vi "VIH HelpGen - Write HTML File - Common - Owning Palette.vi"(5 "HTML Folder":path, 8 "error in":errorcluster, 10 "Owning Palette":cluster{"Name":string, "HTML Path":path}, 11 "HTML in":string) -> (0 "error out":errorcluster, 3 "HTML out":string)   [LabVIEW 2014]
doc: "::: VI Helpeks :::\nCopyright (c) 2000-2026 Konstantin Shifershteyn. All rights reserved."
panel:
  # "VI Helpeks\nCopyright (c) 2012-2026 Konstantin Shifershteyn"
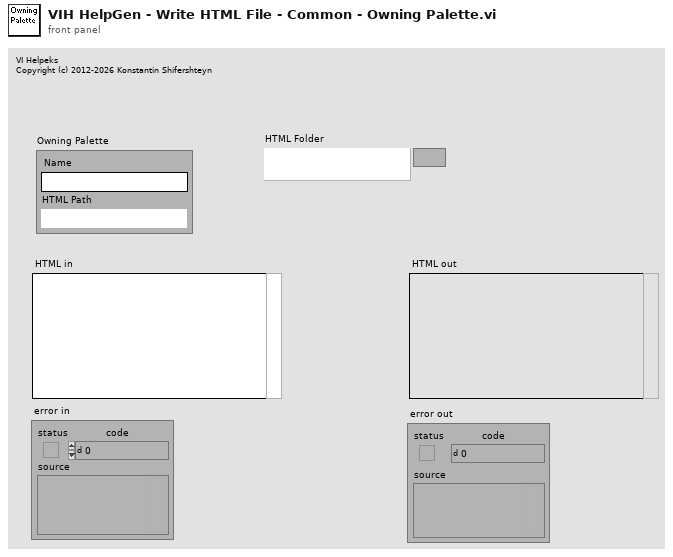
[diagram p1: front panel]
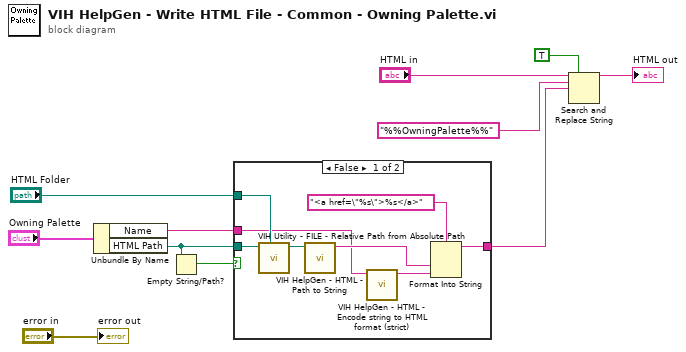
[diagram p0: block diagram]
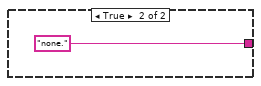
[diagram p2: hidden frame]
diagram:
  n1 = Unbundle By Name("Owning Palette") -> ("Name"=w11:string, "HTML Path"=w10:path)
  n2 = Empty String/Path?(string/path=w10) -> (empty?=w9:bool)
  n3 = case shown="False" w9 {
    tunnel: "HTML Folder" -> [w19 _]
    tunnel: w10 -> [w18 _]
    tunnel: [w15 "none."] -> w2
    tunnel: w11 -> [w13 _]
    frame False {
      n4 = call "VIH Utility - FILE - Relative Path from Absolute Path.vi"("base path (empty: dir of Top VI)"=w19, "Path"=w18) -> ("Rel Path out"=w17:path)  [unwired: 7 in, 2 out]
      n5 = call "VIH HelpGen - HTML - Path to String.vi"("Path"=w17) -> ("String"=w14:string)  [unwired: 10 in]
      n6 = call "VIH HelpGen - HTML - Encode string to HTML format (strict).vi"("string"=w13) -> ("HTML string"=w12:string)  [unwired: 10 in]
      n7 = Format Into String(format string="<a href=\"%s\">%s</a>", w14, w12) -> (resulting string=w15:string)  [unwired: 2 in, 1 out]
    }
    frame True {
    }
  }
  n8 = Search and Replace String(replace all?=TRUE, input string="HTML in", search string="%%OwningPalette%%", replace string=w2) -> (result string=→"HTML out":string)  [unwired: 4 in, 3 out]
  "error out" <- "error in"
